vi "Panel.vi"(11 "DeviceListPanel in":refnum<class "DeviceListPanel.lvclass">) -> ()   [LabVIEW 2020, in "PicoG-App.lvlib" / "DeviceListPanel.lvclass"]
uses:
  DeviceListPanel.lvclass
  C:/Program Files (x86)/National Instruments/LabVIEW 2020/vi.lib/IlluminatedG/IG OOPanel/OOPanel/Panel/Panel.lvclass
  <vilib>/IlluminatedG/IG OOPanel/OOPanel/Panel/Basic UI State.ctl
  DeviceListPanel.lvclass/DeviceListPanel.ctl
  DeviceArrayPanel/DeviceArrayPanel.lvclass
  C:/Program Files (x86)/National Instruments/LabVIEW 2020/vi.lib/IlluminatedG/IG OOPanel/OOPanel/ArrayPanel/ArrayPanel.lvclass
  Device/Device.lvclass
  <vilib>/IlluminatedG/IG OOPanel/OOPanel/Panel/Panel.lvclass
  <vilib>/IlluminatedG/IG OOPanel/OOPanel/OOPanel.lvlib
  <vilib>/IlluminatedG/IG OOPanel/OOPanel/ArrayManager/ArrayManager.lvclass
panel:
  in  "Add":bool
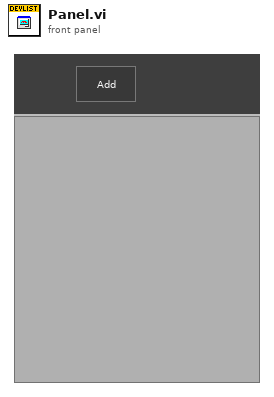
[diagram p1: front panel]
types:
  T1 = typedef "OOPanel.lvlib/Panel.lvclass/Basic UI State.ctl" = enum16{"Init", "Run", "Close"}
  T2 = typedef "PicoG-App.lvlib/DeviceListPanel.lvclass/Inbound Events.ctl" = cluster{"Add Device":refnum<user-event>, "Select Device":refnum<user-event>, "Remove Device":refnum<user-event>, "Refresh Device":refnum<user-event>}
  T3 = typedef "OOPanel.lvlib/Panel.lvclass/Panel Events.ctl" = cluster{"Visbility":refnum<user-event>, "Close":refnum<user-event>}
  T4 = typedef "PicoG-App.lvlib/Device.lvclass/Device Key.ctl" = cluster{"Platform":string, "Board":string, "ID":string}
  T5 = typedef "PicoG-App.lvlib/DeviceListPanel.lvclass/Ref Data.ctl" = cluster{"Map":map{T4, T6}}
  T6 = typedef "PicoG-App.lvlib/DeviceListPanel.lvclass/Device and Panel.ctl" = cluster{"Device":refnum<class "Device.lvclass">, "Panel":refnum<class "DeviceArrayPanel.lvclass">}
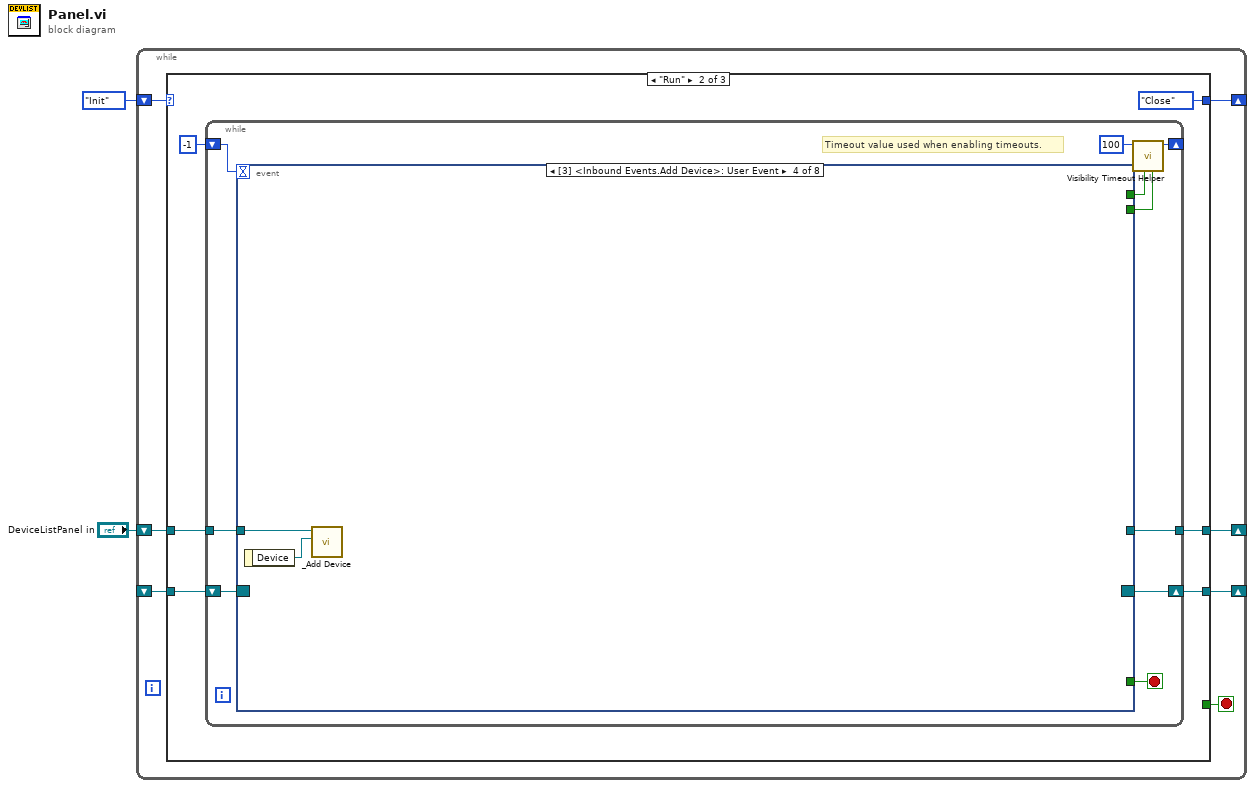
[diagram p0: block diagram]
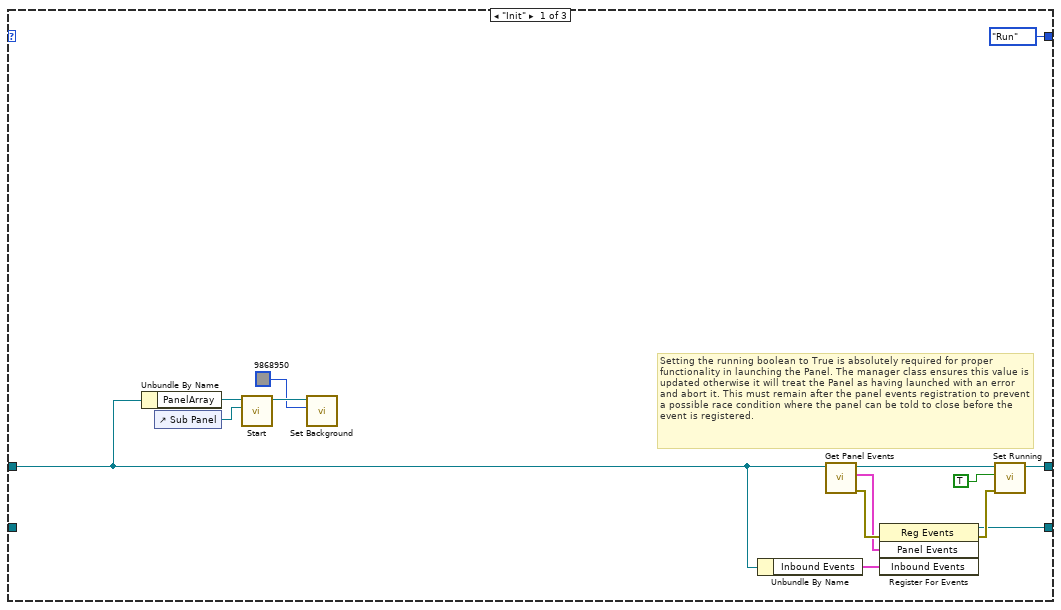
[diagram p2: hidden frame]
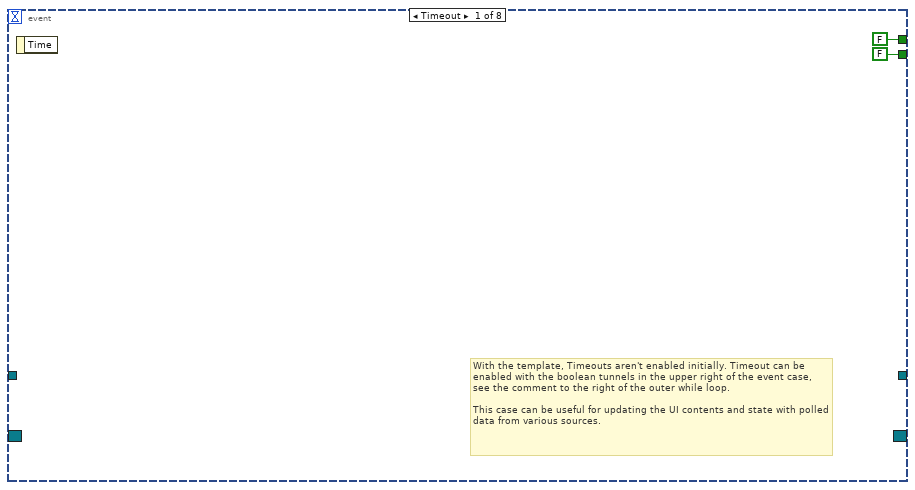
[diagram p3: hidden frame]
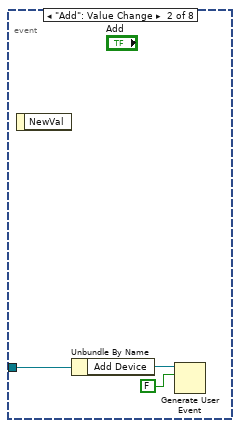
[diagram p4: hidden frame]
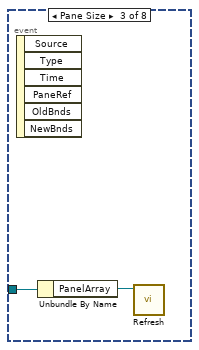
[diagram p5: hidden frame]
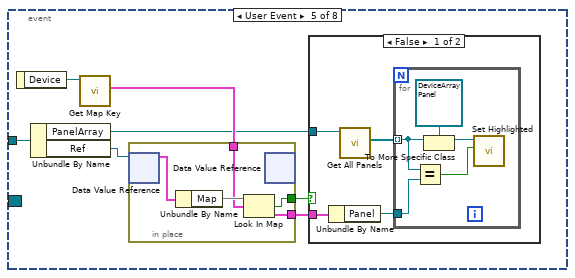
[diagram p6: hidden frame]
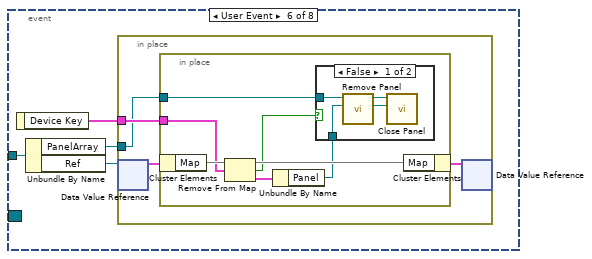
[diagram p8: hidden frame]
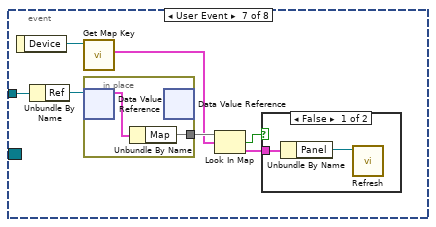
[diagram p10: hidden frame]
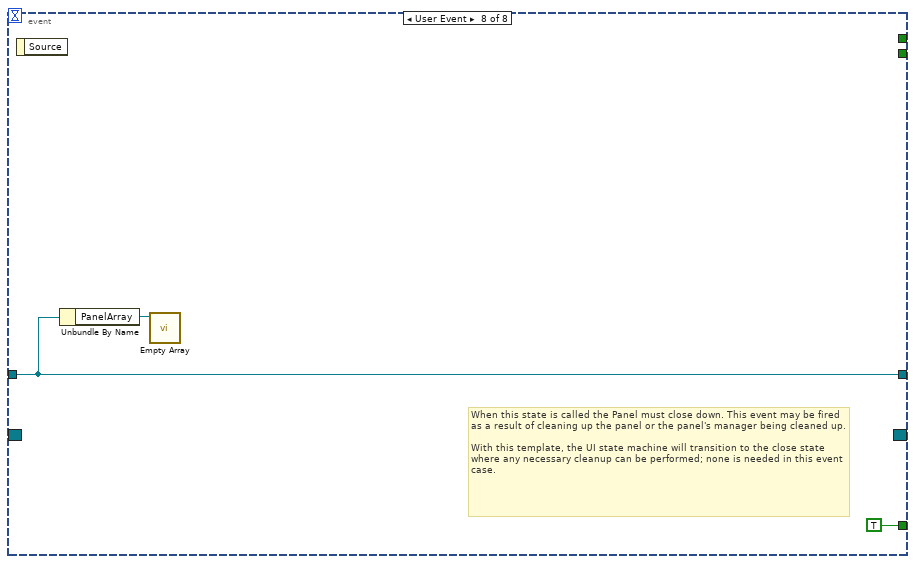
[diagram p12: hidden frame]
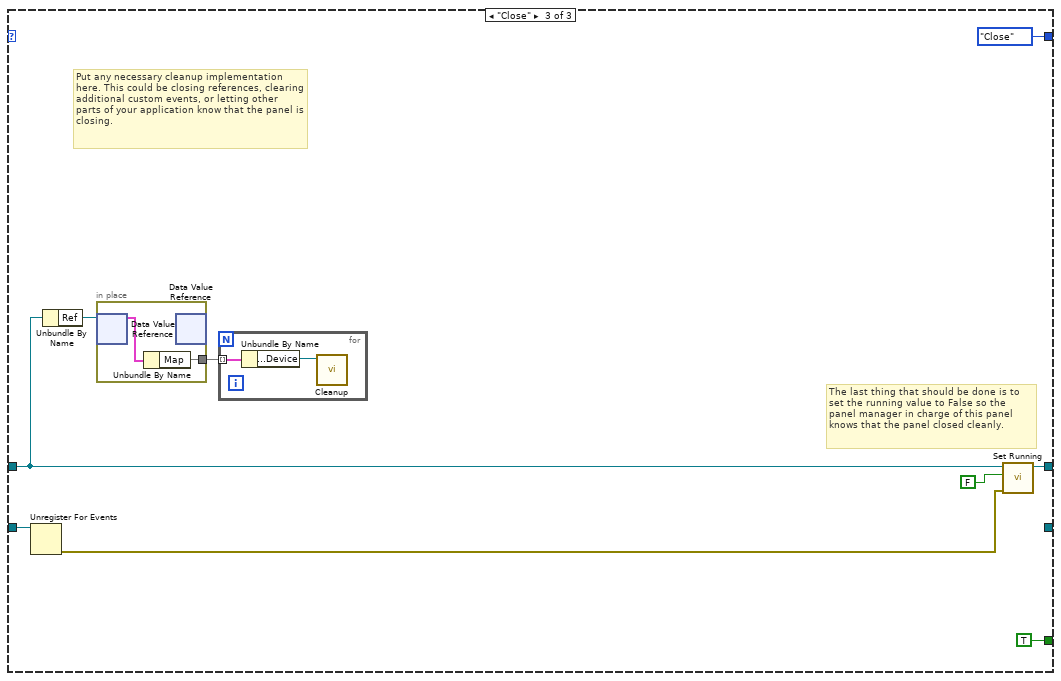
[diagram p13: hidden frame]
diagram:
  n1 = while {
    shift-right: [w8] -> _
    shift-left: _ -> [w9]
    shift-right: [w6] -> _
    shift-left: Basic_UI_State."Init" ("Basic UI State") -> [w7]
    shift-right: [w4] -> _
    shift-left: "DeviceListPanel in" -> [w3]
    stop <- w5 stop-if-true
    n2 = case shown="\"Run\"" w7 {
      tunnel: w9 -> [_ w29 w107]
      tunnel: [w17 w27 _] -> w8
      tunnel: [Basic_UI_State."Run" ("Basic UI State") Basic_UI_State."Close" ("Basic UI State") Basic_UI_State."Close" ("Basic UI State")] -> w6
      tunnel: [_ _ TRUE] -> w5
      tunnel: [w16 w24 w106] -> w4
      tunnel: w3 -> [w14 w25 w104]
      frame "Init" {
        # "Setting the running boolean to True is absolutely required for proper functionality in launching the Panel. The manager class ensures this value is updated otherwise it will treat the Panel as having launched with an error and abort it. This must remain after the panel events registration to prevent a possible race condition where the panel can be told to close before the event is registered."
        n3 = Unbundle By Name(w14) -> ("PanelArray"=w13:refnum<class "ArrayManager.lvclass">)
        n4 = control-ref of="Sub Panel"() -> (w12:refnum<vi>)
        n5 = call <vilib>:"Start.vi"("Container"=w12, "ArrayManager in"=w13) -> ("ArrayManager out"=w11:refnum<class "ArrayManager.lvclass">)  [unwired: 8 in, 1 out]
        n6 = call <vilib>:"Set Background.vi"("Background"=u32 9868950, "ArrayManager in"=w11) -> ()  [unwired: 8 in, 2 out]
        n7 = Unbundle By Name(w14) -> ("Inbound Events"=w15:T2)
        n8 = call <vilib>:"Get Panel Events.vi"("Panel in"=w14) -> ("error out"=w23:errorcluster, "Panel Events"=w19:T3, "Panel out"=w20:refnum<class "DeviceListPanel.lvclass">)  [unwired: 8 in]
        n9 = register-events(error in=w23, w19, w15) -> (reference out=w17:refnum<event-registration>, error out=w21:errorcluster)  [unwired: 1 in]
        n10 = call <vilib>:"Set Running.vi"("error in (no error)"=w21, "Running"=TRUE, "Panel in"=w20) -> ("Panel out"=w16:refnum<class "DeviceListPanel.lvclass">)  [unwired: 7 in, 1 out]
      }
      frame "Run" {
        n11 = while {
          shift-right: [w35] -> w27
          shift-left: w29 -> [w36]
          shift-right: [w38] -> _
          shift-left: -1 ("Timeout") -> [w37]
          tunnel: w25 -> [w31]
          tunnel: [w30] -> w24
          stop <- w32 stop-if-true
          # "Timeout value used when enabling timeouts."
          n12 = event shown="[3] <Inbound Events.Add Device>: User Event" {
            selector: w36 -> [_ _ _ _ _ _ _ _]
            dyn-events: [_ _ _ _ _ _ _ _] -> w35
            timeout: w37 -> [_ _ _ _ _ _ _ _]
            tunnel: [FALSE _ _ _ _ _ _ _] -> w34
            tunnel: [FALSE _ _ _ _ _ _ _] -> w33
            tunnel: [_ _ _ _ _ _ _ TRUE] -> w32
            tunnel: w31 -> [_ w44 w46 w48 w54 w73 w94 w101]
            tunnel: [_ _ _ _ _ _ _ w101] -> w30
            event Timeout {
              # "With the template, Timeouts aren't enabled initially. Timeout can be enabled with the boolean tunnels in the upper right of the event case, see the comment to the right of the outer while loop.\n\nThis case can be useful for updating the UI contents and state with polled data from various sources."
              n13 = event-data() -> ()  [unwired: 1 in, 1 out]
            }
            event "Add": Value Change {
              n14 = event-data() -> ()  [unwired: 1 in, 1 out]
              n15 = Unbundle By Name(w44) -> ("Add Device"=w43:refnum<user-event>)
              n16 = Generate User Event(user event=w43, event data cluster=FALSE ("event data")) -> ()  [unwired: 2 in, 2 out]
            }
            event Pane Size {
              n17 = event-data() -> ()  [unwired: 1 in, 6 out]
              n18 = Unbundle By Name(w46) -> ("PanelArray"=w45:refnum<class "ArrayManager.lvclass">)
              n19 = call <vilib>:"Refresh.vi"("ArrayManager in"=w45) -> ()  [unwired: 9 in, 2 out]
            }
            event User Event {
              n20 = event-data() -> ("Device"=w47:refnum<class "Device.lvclass">)  [unwired: 1 in]
              n21 = call "_Add Device.vi"("Device"=w47, "DeviceListPanel in"=w48) -> ()  [unwired: 8 in, 2 out]
            }
            event User Event {
              n22 = event-data() -> ("Device"=w53:refnum<class "Device.lvclass">)  [unwired: 1 in]
              n23 = Unbundle By Name(w54) -> ("PanelArray"=w49:refnum<class "ArrayManager.lvclass">, "Ref"=w55:refnum<data-value>)
              n24 = call "Get Map Key.vi"("Device in"=w53) -> ("Key"=w52:T4)  [unwired: 8 in, 2 out]
              n25 = in-place {
                in-place-border: w52 -> [w67]
                in-place-border: [w66] -> w51
                in-place-border: [w65] -> w50
                n26 = in-place-dvr #1(w55) -> (w69:T5)  [unwired: 1 out]
                n27 = Unbundle By Name(w69) -> ("Map"=w68:map{T4, T6})
                n28 = Look In Map(map=w68, key=w67) -> (key not found?=w66:bool, value=w65:T6)  [unwired: 1 in]
                n29 = in-place-dvr #1() -> ()  [unwired: 1 in, 2 out]
              }
              n30 = case shown="False" w51 {
                tunnel: w50 -> [w59 _]
                tunnel: w49 -> [w58 _]
                frame False {
                  n31 = Unbundle By Name(w59) -> ("Panel"=w56:refnum<class "DeviceArrayPanel.lvclass">)
                  n32 = call <vilib>:"Get All Panels.vi"("PanelArray in"=w58) -> ("Panels"=w57:refnum<class "ArrayPanel.lvclass">[])  [unwired: 8 in, 2 out]
                  n33 = for {
                    tunnel: w57 -> [w63] mode=indexing
                    tunnel: w56 -> [w64]
                    n34 = Equal?(x=w63, y=w64) -> (x = y?=w60:bool)
                    n35 = To More Specific Class(target class=refnum<class "DeviceArrayPanel.lvclass"> refnum ("PicoG-App.lvlib:DeviceArrayPanel.lvclass"), reference=w63) -> (specific class reference=w61:refnum<class "DeviceArrayPanel.lvclass">)  [unwired: 1 in, 1 out]
                    n36 = call "Set Highlighted.vi"("Highlighted"=w60, "DeviceArrayPanel in"=w61) -> ()  [unwired: 8 in, 2 out]
                  }
                }
                frame True {
                  # "#ERROR?"
                }
              }
            }
            event User Event {
              n37 = event-data() -> ("Device Key"=w70:T4)  [unwired: 1 in]
              n38 = Unbundle By Name(w73) -> ("PanelArray"=w71:refnum<class "ArrayManager.lvclass">, "Ref"=w72:refnum<data-value>)
              n39 = in-place {
                in-place-border: w71 -> [w75]
                in-place-border: w70 -> [w76]
                n40 = in-place-dvr #2(w72) -> (w77:T5)  [unwired: 1 out]
                n41 = in-place {
                  in-place-border: w76 -> [w83]
                  in-place-border: w75 -> [w80]
                  n42 = in-place-cluster #3(w77) -> ("Map"=w84:map{T4, T6})
                  n43 = Remove From Map(10:w83, 11:w84) -> (1:w79:T6, 2:w81:bool, 3:w82:map{T4, T6})
                  n44 = Unbundle By Name(w79) -> ("Panel"=w78:refnum<class "DeviceArrayPanel.lvclass">)
                  n45 = case shown="False" w81 {
                    tunnel: w80 -> [w88 _]
                    tunnel: w78 -> [w87 _]
                    frame False {
                      n46 = call <vilib>:"Remove Panel.vi"("Panel in"=w87, "ArrayManager in"=w88) -> ("Panel"=w85:refnum<class "ArrayPanel.lvclass">, "ArrayManager out"=w86:refnum<class "ArrayManager.lvclass">)  [unwired: 7 in, 1 out]
                      n47 = call <vilib>:"Close Panel.vi"("ArrayPanel"=w85, "ArrayManager in"=w86) -> ()  [unwired: 8 in, 2 out]
                    }
                    frame True {
                    }
                  }
                  n48 = in-place-cluster #3("Map"=w82) -> (w74:T5)
                }
                n49 = in-place-dvr #2(w74) -> ()  [unwired: 2 out]
              }
            }
            event User Event {
              n50 = event-data() -> ("Device"=w92:refnum<class "Device.lvclass">)  [unwired: 1 in]
              n51 = Unbundle By Name(w94) -> ("Ref"=w95:refnum<data-value>)
              n52 = call "Get Map Key.vi"("Device in"=w92) -> ("Key"=w91:T4)  [unwired: 8 in, 2 out]
              n53 = in-place {
                in-place-border: [w98] -> w93
                n54 = in-place-dvr #4(w95) -> (w99:T5)  [unwired: 1 out]
                n55 = Unbundle By Name(w99) -> ("Map"=w98:map{T4, T6})
                n56 = in-place-dvr #4() -> ()  [unwired: 1 in, 2 out]
              }
              n57 = Look In Map(map=w93, key=w91) -> (key not found?=w90:bool, value=w89:T6)  [unwired: 1 in]
              n58 = case shown="False" w90 {
                tunnel: w89 -> [w97 _]
                frame False {
                  n59 = Unbundle By Name(w97) -> ("Panel"=w96:refnum<class "DeviceArrayPanel.lvclass">)
                  n60 = call <vilib>:"Refresh.vi"("DeviceArrayPanel in"=w96) -> ()  [unwired: 9 in, 2 out]
                }
                frame True {
                }
              }
            }
            event User Event {
              # "When this state is called the Panel must close down. This event may be fired as a result of cleaning up the panel or the panel's manager being cleaned up.\n\nWith this template, the UI state machine will transition to the close state where any necessary cleanup can be performed; none is needed in this event case."
              n61 = event-data() -> ()  [unwired: 1 in, 1 out]
              n62 = Unbundle By Name(w101) -> ("PanelArray"=w100:refnum<class "ArrayManager.lvclass">)
              n63 = call <vilib>:"Empty Array.vi"("ArrayManager in"=w100) -> ()  [unwired: 9 in, 2 out]
            }
          }
          n64 = call <vilib>:"Visibility Timeout Helper.vi"("Update?"=w33, "Use Timeout?"=w34, "Visible Timeout mS"=100) -> ("Timeout"=w38:i32)  [unwired: 8 in]
        }
      }
      frame "Close" {
        # "Put any necessary cleanup implementation here. This could be closing references, clearing additional custom events, or letting other parts of your application know that the panel is closing."
        # "The last thing that should be done is to set the running value to False so the panel manager in charge of this panel knows that the panel closed cleanly."
        n65 = Unregister For Events(event registration refnum=w107) -> (error out=w109:errorcluster)  [unwired: 1 in]
        n66 = Unbundle By Name(w104) -> ("Ref"=w105:refnum<data-value>)
        n67 = in-place {
          in-place-border: [w114] -> w103
          n68 = in-place-dvr #5(w105) -> (w115:T5)  [unwired: 1 out]
          n69 = Unbundle By Name(w115) -> ("Map"=w114:map{T4, T6})
          n70 = in-place-dvr #5() -> ()  [unwired: 1 in, 2 out]
        }
        n71 = for {
          tunnel: w103 -> [w113] mode=indexing
          n72 = Unbundle By Name(w113) -> ("Value Type.Device"=w112:refnum<class "Device.lvclass">)
          n73 = call "Cleanup.vi"("Device in"=w112) -> ()  [unwired: 10 in, 1 out]
        }
        n74 = call <vilib>:"Set Running.vi"("error in (no error)"=w109, "Running"=FALSE, "Panel in"=w104) -> ("Panel out"=w106:refnum<class "DeviceListPanel.lvclass">)  [unwired: 7 in, 1 out]
      }
    }
  }
